vi "I2C Write.vi"(8 "error in (no error)":errorcluster, 10 "Values":u8[](array[numeric]), 11 "I2C Device":T1) -> (0 "error out":errorcluster, 3 "I2C Device out":T1)   [LabVIEW 2020, in "wiringPi.lvlib"]
doc: "<b>_______________________________________________________________</b>\n** Author: Juan José Villacorta\n** LabVIEW wrapper for C library <b> wiringPi </b>,\n** https://github.com/WiringPi/WiringPi\n<b>_______________________________________________________________</b>\n/*\n * Write a block of data to a register on the device\n**********************************************************************************\n*/"
uses:
  wiringPi.lvlib
  Type Defs/I2C Device.ctl
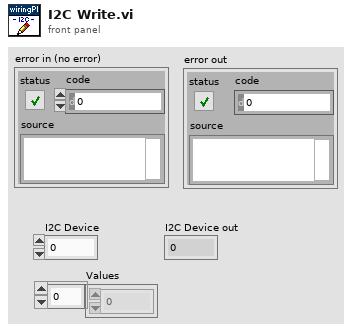
[diagram p1: front panel]
types:
  T1 = typedef "wiringPi.lvlib/I2C Device.ctl" = i32
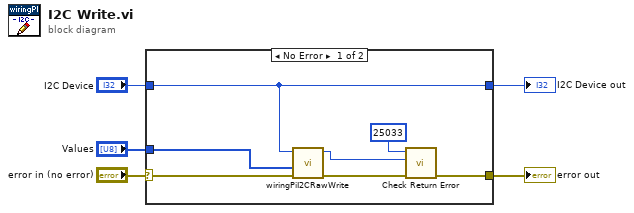
[diagram p0: block diagram]
diagram:
  n1 = case shown="No Error" "error in (no error)" {
    selector: "error in (no error)" -> [w11 w14]
    tunnel: [w12 w14] -> w4
    tunnel: "I2C Device" -> [w9 w13]
    tunnel: [w9 w13] -> w3
    tunnel: "Values" -> [w6 _]
    frame No Error {
      n2 = call "wiringPiI2CRawWrite.vi"("error in (no error)"=w11, "values"=w6, "devID"=w9) -> ("error out"=w10:errorcluster, "return"=w8:i32)  [unwired: 7 in]
      n3 = call "Check Return Error.vi"("error in (no error)"=w10, "Return code"=w8, "Error number"=25033) -> ("error out"=w12:errorcluster)  [unwired: 8 in]
    }
    frame Error {
    }
  }
  "error out" <- w4
  "I2C Device out" <- w3
